vi "CSM - MassData Data Type String.vi"(7 "error in (no error)":errorcluster, 9 "MassData Argument":string) -> (1 "error out":errorcluster, 2 "Data Type String":string, 3 "MassData Argument (dup)":string)   [LabVIEW 2017, in "CSM MassData Parameter Support.lvlib"]
doc: "Extracts the data type string from a Massdata argument.\n\n\n> [!NOTE] <b>CSM Massdata Argument Format</b>\n>\n> A typical Massdata data format is: `<MassData>Start:8057;Size:4004;DataType:1D I32`.\n>\n> where:\n> - `Start`: The starting address of the data in memory.\n> - `Size`: The size of the data in bytes.\n> - `DataType(optional)`: The type of the data, defined by the CSM Data Type String VI.\n\n\n-- <b>Controls</b> --\n- <b>MassData Argument</b>: Input Massdata argument.\n\n-- <b>Indicators</b> --\n- <b>MassData Argument(dup)</b>: A copy of the input Massdata argument.\n- <b>Data Type String</b>: The parsed data type string."
uses:
  CSM MassData Parameter Support.lvlib
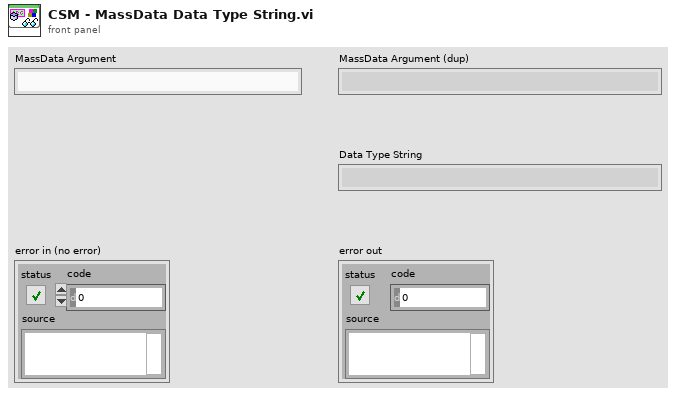
[diagram p1: front panel]
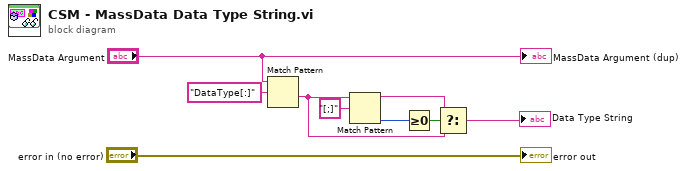
[diagram p0: block diagram]
diagram:
  n1 = Match Pattern(string="MassData Argument", regular expression="DataType[:]") -> (after substring=w2:string)  [unwired: 1 in, 3 out]
  n2 = Match Pattern(string=w2, regular expression="[;]") -> (before substring=w3:string, offset past match=w5:i32)  [unwired: 1 in, 2 out]
  n3 = Greater Or Equal To 0?(x=w5) -> (x >= 0?=w4:bool)
  n4 = Select(t=w3, s=w4, f=w2) -> (s? t:f=→"Data Type String":string)
  "MassData Argument (dup)" <- "MassData Argument"
  "error out" <- "error in (no error)"
